vi "CSE routine - Error Handler.vi"(5 "nesting level":i32=1, 6 "error in":errorcluster, 8 "exec status":i32, 9 "CSE RefNum":T1) -> (0 "error out":errorcluster, 2 "dup exec status":i32, 3 "dup CSE RefNum":T1)   [LabVIEW 2021]
doc: "::: CalcExpress Toolkit :::\nCopyright (c) 2000-2026 Konstantin Shifershteyn. All rights reserved."
uses:
  CSE Instance RefNum.ctl
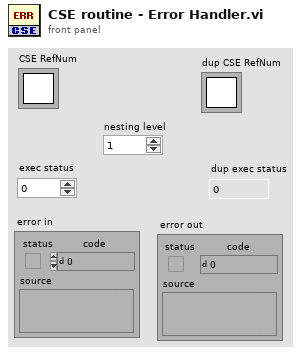
[diagram p1: front panel]
types:
  T1 = typedef "CSE Instance RefNum.ctl" = refnum<k1>
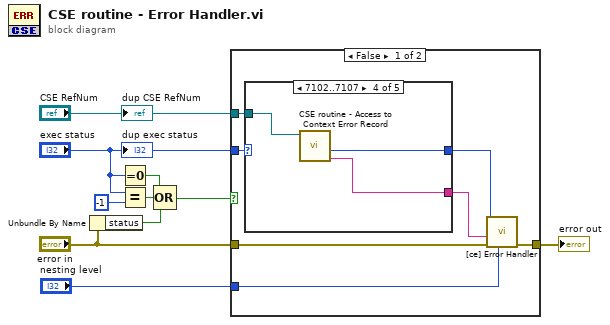
[diagram p0: block diagram]
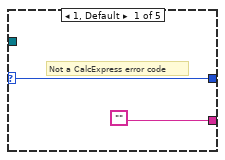
[diagram p2: hidden frame]
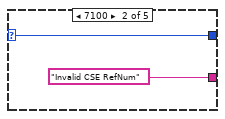
[diagram p3: hidden frame]
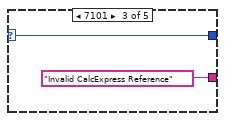
[diagram p4: hidden frame]
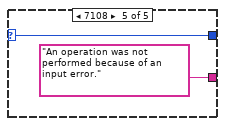
[diagram p5: hidden frame]
diagram:
  n1 = Unbundle By Name("error in") -> ("status"=w6:bool)
  n2 = Equal To 0?(x="exec status") -> (x = 0?=w8:bool)
  n3 = Equal?(x="exec status", y=-1) -> (x = y?=w7:bool)
  n4 = Compound Arithmetic op=OR(w8, w7, w6) -> (w5:bool)
  n5 = case shown="False" w5 {
    tunnel: "exec status" -> [w17 _]
    tunnel: "error in" -> [w15 w29]
    tunnel: [w13 w29] -> w10
    tunnel: "CSE RefNum" -> [w12 _]
    tunnel: "nesting level" -> [w11 _]
    frame False {
      n6 = case shown="7102..7107" w17 {
        selector: w17 -> [w19 w20 w22 _ w28]
        tunnel: ["" ("Empty String Constant") "Invalid CSE RefNum" "Invalid CalcExpress Reference" w24 "An operation was not performed because of an input error." ("error message out")] -> w14
        tunnel: [w19 w20 w22 w26 w28] -> w16
        tunnel: w12 -> [_ _ _ w25 _]
        frame 1, Default {
          # "Not a CalcExpress error code"
        }
        frame 7100 {
        }
        frame 7101 {
        }
        frame 7102..7107 {
          n7 = call "CSE routine - Access to Context Error Record.vi"("CSE RefNum"=w25) -> ("error message out"=w24:string, "error code out"=w26:i32)  [unwired: 6 in, 3 out]
        }
        frame 7108 {
        }
      }
      n8 = call "[ce] Error Handler.vi"("nesting level"=w11, "error in"=w15, "error reason"=w14, "error code"=w16) -> ("error out"=w13:errorcluster)  [unwired: 6 in, 1 out]
    }
    frame True {
    }
  }
  "error out" <- w10
  "dup CSE RefNum" <- "CSE RefNum"
  "dup exec status" <- "exec status"
